vi "G-Uart_config-init.vi"(8 "error in (no error)":errorcluster caption="错误输入（无错误）", 10 "路径":path, 11 "G-Uart-Class 输入":refnum<class "G-Uart-Class.lvclass">) -> (0 "error out":errorcluster caption="错误输出", 3 "G-Uart-Class 输出":refnum<class "G-Uart-Class.lvclass">)   [LabVIEW 2025, in "G-Uart-Class.lvclass"]
uses:
  G-Uart-Class.lvclass
  <vilib>/Instr/_visa.llb/VISA Set IO Buffer Mask.ctl
panel:
  # "欢迎使用小高的串口类"
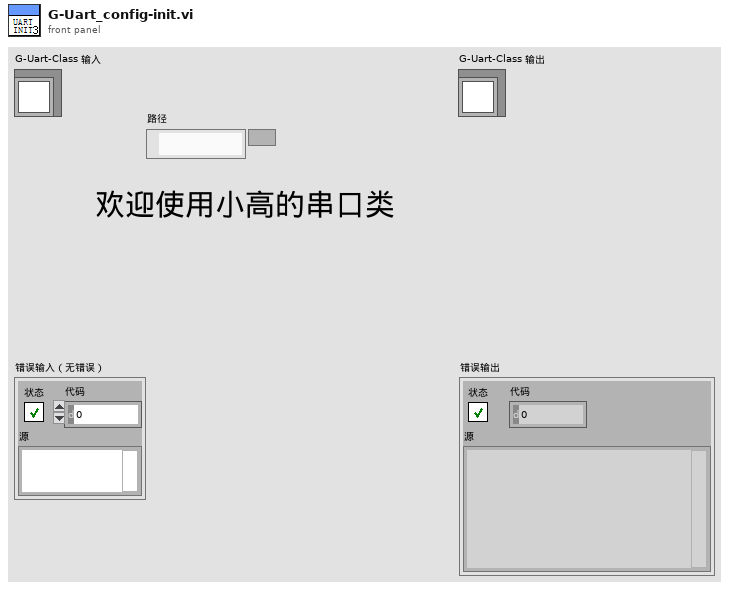
[diagram p1: front panel]
types:
  T1 = typedef "VISA Set IO Buffer Mask.ctl" = u16
  T2 = cluster{"VISA resource name":refnum<visa-resource-name>, "baud rate (9600)":u32, "data bits (8)":u16, "parity (0:none)":enum16{"None", "Odd", "Even", "Mark", "Space"}, "stop bits (10: 1 bit)":u16, "flow control (0:none)":u16, "timeout (10sec)":u32, "Enable Termination\nChar (T)":bool, "termination char\n(0xA = '\\n' = LF) ":u8}[]
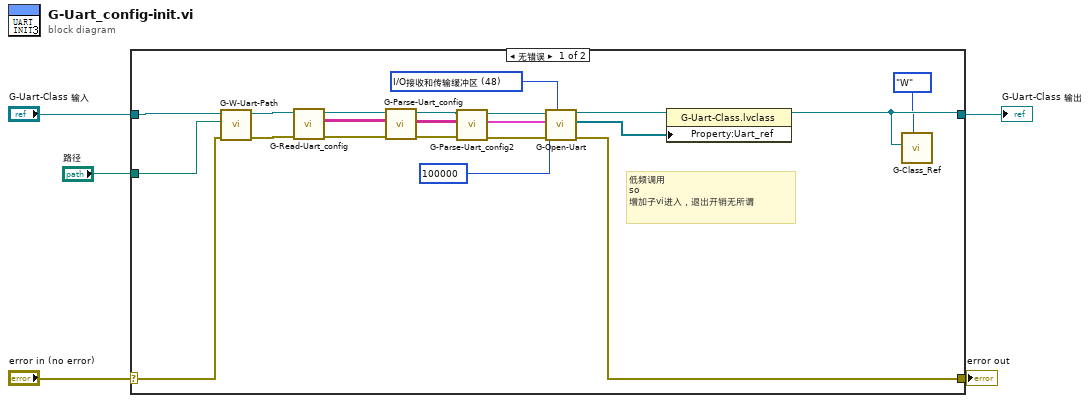
[diagram p0: block diagram]
diagram:
  n1 = case shown="无错误" "error in (no error)" {
    selector: "error in (no error)" -> [w24 w28]
    tunnel: [w13 w28] -> w4
    tunnel: [w7 w27] -> w2
    tunnel: "G-Uart-Class 输入" -> [w26 w27]
    tunnel: "路径" -> [w25 _]
    frame No Error {
      w9 = T1 48 items=["I/O接收缓冲区"=16, "I/O传输缓冲区"=32, "I/O接收和传输缓冲区"=48] ("Mask")
      # "低频调用\nso\n增加子vi进入，退出开销无所谓"
      n2 = call-dynamic "G-W-Uart-Path.vi"("error in (no error)"=w24, "路径"=w25, "G-Uart-Class输入"=w26) -> ("error out"=w20:errorcluster, "G-Uart-Class输出"=w23:refnum<class "G-Uart-Class.lvclass">)  [unwired: 7 in]
      n3 = call-dynamic "G-Read-Uart_config.vi"("error in (no error)"=w20, "G-Uart-Class 输入"=w23) -> ("error out"=w19:errorcluster, "data"=w21:string[][], "G-Uart-Class 输出"=w22:refnum<class "G-Uart-Class.lvclass">)  [unwired: 7 in]
      n4 = call-dynamic "G-Parse-Uart_config.vi"("error in (no error)"=w19, "Data"=w21, "G-Uart-Class 输入"=w22) -> ("error out"=w17:errorcluster, "配置数组"=w16:string[][], "G-Uart-Class 输出"=w18:refnum<class "G-Uart-Class.lvclass">)  [unwired: 6 in]
      n5 = call-dynamic "G-Parse-Uart_config2.vi"("error in (no error)"=w17, "配置数组"=w16, "G-Uart-Class 输入"=w18) -> ("error out"=w14:errorcluster, "数组"=w12:T2, "G-Uart-Class 输出"=w15:refnum<class "G-Uart-Class.lvclass">)  [unwired: 6 in]
      n6 = call-dynamic "G-Open-Uart.vi"("Mask"=w9, "error in (no error)"=w14, "大小(4096)"=u32 100000, "数组"=w12, "G-Uart-Class 输入"=w15) -> ("error out"=w13:errorcluster, "数组 2"=w10:refnum<visa-resource-name>[], "G-Uart-Class 输出"=w11:refnum<class "G-Uart-Class.lvclass">)  [unwired: 4 in]
      n7 = property class="G-Uart-Class.lvclass"(reference=w11, "Property:Uart_ref"=w10) -> (reference out=w7:refnum<class "G-Uart-Class.lvclass">)  [unwired: 1 in, 1 out]
      n8 = call "G-Class_Ref.vi"("枚举"=enum16{"R", "W"}."W", "句柄输入"=w7) -> ()  [unwired: 9 in, 1 out]
    }
    frame Error {
    }
  }
  "error out" <- w4
  "G-Uart-Class 输出" <- w2
